vi "properties.set.vi"(8 "error in":errorcluster, 10 "properties":map{string, string}(c390), 11 "asset in":refnum<class "asset.lvclass">) -> (0 "error out":errorcluster, 3 "asset out":refnum<class "asset.lvclass">)   [LabVIEW 2020, in "asset.lvclass"]
uses:
  asset.lvclass
  asset.lvclass/asset.ctl
  Nominal Client/Nominal Client.lvclass/Nominal Client.ctl
  Nominal Client/error.vi
  Nominal Client/trace.payload_sent.vi
  Nominal Client/trace.payload_received.vi
  Nominal Client/create.authorization_header.vi
  Nominal Client/error.vi/859f8e04-e495-489b-b5b4-7ac163f56130.vi
  Nominal Client/trace.calling_method.vi
  <vilib>/JDP Science/JDP Science Common Utilities/Trim Whitespace__JDP.vi
  <vilib>/AdvancedString/1D String Array to Delimited String.vi
  Nominal Client/api_token.get.vi
  <vilib>/JDP Science/JSONtext/support/Format JSON Object.vi
  <vilib>/Utility/libraryn.llb/Get File Extension.vi
  Nominal Client/log_file.write.vi
  <vilib>/JDP Science/JSONtext/Get all Object Items.vi
  <vilib>/Utility/error.llb/Error Cluster From Error Code.vi
  <vilib>/JDP Science/JSONtext/JSON text to Variant.vi
  <vilib>/JDP Science/JSONtext/LVClass Serializer/JSONtext LVClass Serializer.lvclass
  <vilib>/addons/_JKI.lib/REST Client/classes/Response Headers/Response Headers.lvclass
  nominal types/properties/properties.lvclass
  <vilib>/addons/_JKI.lib/REST Client/classes/REST Client/REST Client.lvclass
  Nominal Client/Nominal Client.lvclass
  <vilib>/JDP Science/JSONtext/JSONtext.lvlib
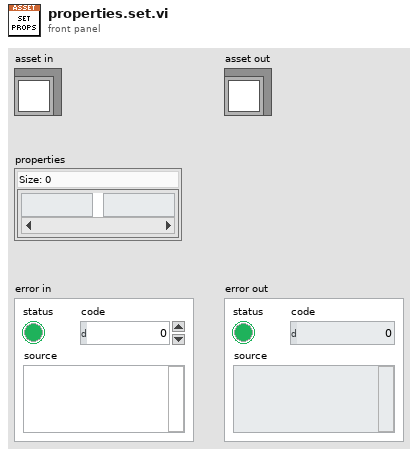
[diagram p1: front panel]
types:
  T1 = typedef "dataScopes.lvlib/links.ctl" = cluster{"URL":string, "Title":string}[]
  T2 = typedef "dataScopes.lvlib/data_scopes.ctl" = T3[]
  T3 = typedef "dataScopes.lvlib/data_scope.ctl" = cluster{"dataScopeName":string, "dataSource":T4, "seriesTags":map{string, string}, "offset":T6}
  T4 = typedef "dataScopes.lvlib/data_source.ctl" = cluster{"type":T5, "rid":string}
  T5 = typedef "dataScopes.lvlib/type.ctl" = enum16{"dataset", "connection", "logSet", "video"}
  T6 = typedef "dataScopes.lvlib/offset.ctl" = cluster{"seconds":i32, "nanos":i32, "picos":i32}
  T7 = cluster{"rid":string, "title":string, "properties":refnum<class "properties.lvclass">, "labels":refnum<class "labels.lvclass">, "Links":T1, "datascopes":T2, "createdAt":timestamp, "updatedAt":timestamp, "attachments":refnum<class "labels.lvclass">, "isStaged":bool, "isArchived":bool, "description":string, "createdBy":string, "type":string}
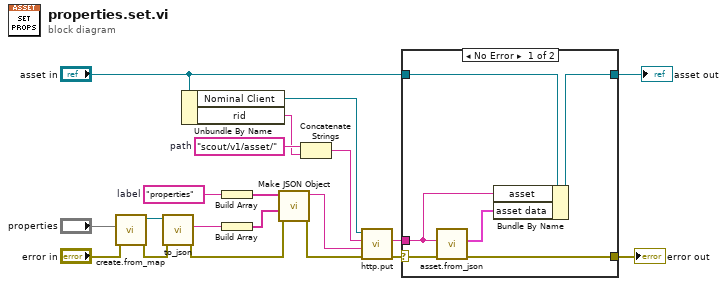
[diagram p0: block diagram]
diagram:
  w8 = "properties"  # label
  w19 = "scout/v1/asset/"  # path
  n1 = call "create.from_map.vi"("error in"="error in", "properties"="properties") -> ("error out"=w2:errorcluster, "properties out"=w3:refnum<class "properties.lvclass">)  [unwired: 8 in]
  n2 = call-dynamic "to_json.vi"("error in"=w2, "properties in"=w3) -> ("error out"=w5:errorcluster, "json"=w11:string)  [unwired: 6 in, 2 out]
  n3 = Unbundle By Name("asset in") -> ("Nominal Client"=w20:refnum<class "Nominal Client.lvclass">, "rid"=w17:string)
  n4 = Build Array(w8) -> (w9:string[])
  n5 = Build Array(w11) -> (w10:string[])
  n6 = call <vilib>:"Make JSON Object.vi"("error in (no error)"=w5, "JSON Items"=w10, "Item Names"=w9) -> ("error out"=w6:errorcluster, "<JSON>"=w7:string)  [unwired: 7 in]
  n7 = Concatenate Strings(w19, w17) -> (w18:string)
  n8 = call "http.put.vi"("error in"=w6, "Body"=w7, "Path"=w18, "Nominal Client in"=w20) -> ("error out"=w16:errorcluster, "Response"=w13:string)  [unwired: 4 in, 2 out]
  n9 = case shown="No Error" w16 {
    selector: w16 -> [w26 w28]
    tunnel: [w25 w28] -> w15
    tunnel: "asset in" -> [w24 w27]
    tunnel: w13 -> [w22 _]
    tunnel: [w21 w27] -> w12
    frame No Error {
      n10 = call "asset.from_json.vi"("error in"=w26, "asset"=w22) -> ("error out"=w25:errorcluster, "Asset Data"=w23:T7)  [unwired: 8 in]
      n11 = Bundle By Name(cluster=w24, "asset"=w22, "asset data"=w23) -> (w21:refnum<class "asset.lvclass">)
    }
    frame Error {
    }
  }
  "asset out" <- w12
  "error out" <- w15
